vi "Read MR8888 File.vi"(11 "Path":path=path "D:/同步空间/曲线生成/原始曲线/8、记录仪MR8888--AUTO0001.csv") -> (3 "Data Series":T1[](array[typedef]))   [LabVIEW 2020, in "Data Viewer.lvlib"]
uses:
  Data Viewer.lvlib
  Data Serie--cluster.ctl
  File Type--enum.ctl
  45ada8d8-9367-42c1-a51c-dab00799f42c.vi
  4505f498-e49c-4e88-80e6-bc2a5fe8a2a1.vi
  1e224d21-03f6-4504-93f9-5a21471556d5.vi
  2c9b7013-6681-49c9-91fb-dfb68bc23b96.vi
  <vilib>/Utility/file.llb/Read Delimited Spreadsheet (string).vi
  <vilib>/Comparison/Equal/Equal Functor/Equal Functor.lvclass
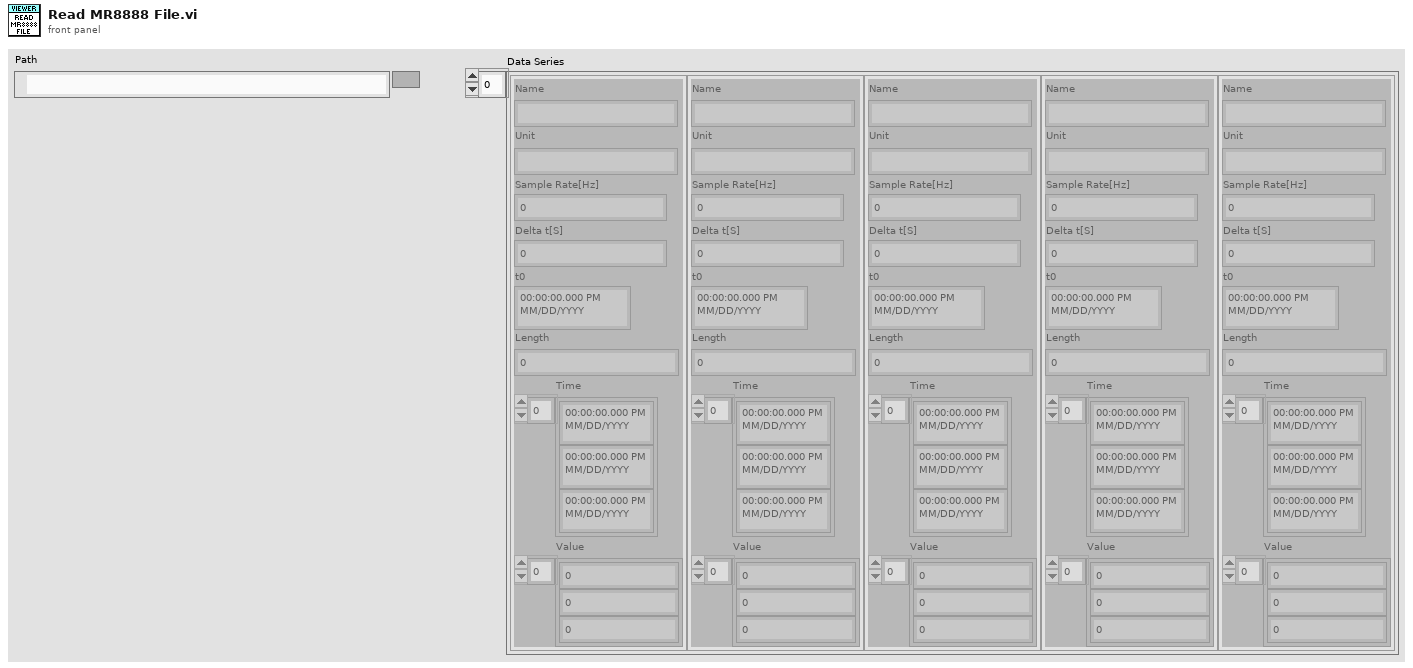
[diagram p1: front panel]
types:
  T1 = typedef "Data Viewer.lvlib/Data Serie--cluster.ctl" = cluster{"Name":string, "Unit":string, "Sample Rate[Hz]":dbl, "Delta t[S]":dbl, "t0":timestamp, "Length":i32, "Time":timestamp[], "Value":dbl[]}
  T2 = typedef "Data Viewer.lvlib/File Type--enum.ctl" = enum16{"伟思环境箱", "增达环境箱", "广五所环境箱", "无纸记录仪", "帕捷SA00339", "记录仪840", "记录仪8400", "记录仪MR888", "*.csv"}
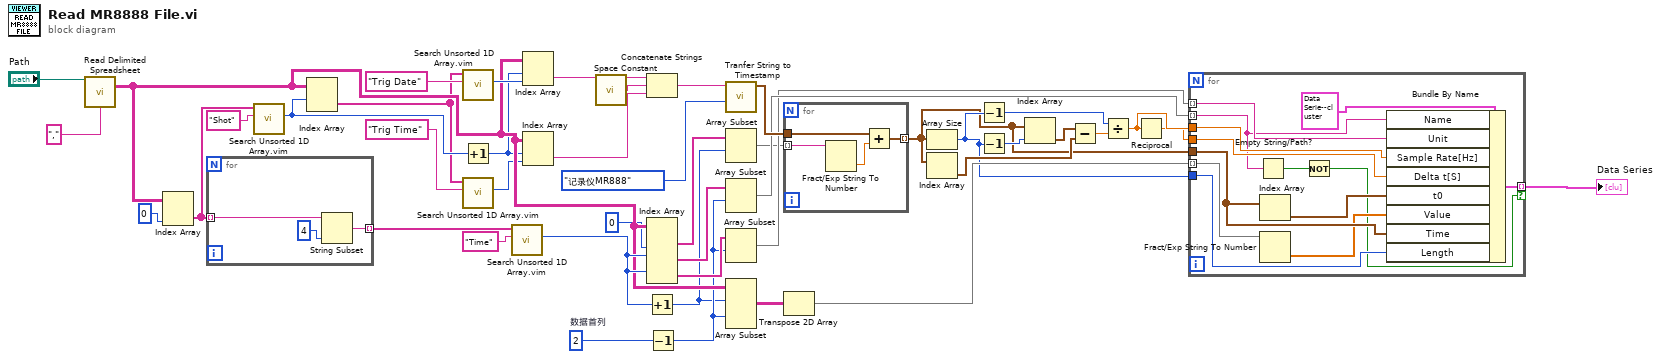
[diagram p0: block diagram]
diagram:
  w18 = 2  # 数据首列
  n1 = call-poly <vilib>:"Read Delimited Spreadsheet.vi"("file path (dialog if empty)"="Path", "delimiter (\\t)"="," ("delimiter (\\t)")) -> ("all rows"=w31:string[][])  [unwired: 8 in, 5 out]
  n2 = Index Array(array=w31, index (col)=0 ("disabled index (col)")) -> (element=w36:string[])  [unwired: 1 in]
  n3 = for {
    tunnel: w36 -> [w47] mode=indexing
    tunnel: [w45] -> w35 mode=indexing
    n4 = String Subset(string=w47, length (rest)=4 ("length (rest)")) -> (substring=w45:string)  [unwired: 1 in]
  }
  n5 = call "Search Unsorted 1D Array.vim"("element"="Shot", "unsorted 1D array"=w36) -> ("index of element"=w33:i32)  [unwired: 9 in]
  n6 = Index Array(array=w31, index (row)=w33) -> (element=w28:string[])  [unwired: 1 in]
  n7 = call "Search Unsorted 1D Array.vim"("element"="Trig Date", "unsorted 1D array"=w28) -> ("index of element"=w32:i32)  [unwired: 9 in]
  n8 = Increment(x=w33) -> (x+1=w30:i32)
  n9 = call "Search Unsorted 1D Array.vim"("element"="Trig Time", "unsorted 1D array"=w28) -> ("index of element"=w27:i32)  [unwired: 9 in]
  n10 = call "Search Unsorted 1D Array.vim"("element"="Time", "unsorted 1D array"=w35) -> ("index of element"=w40:i32)  [unwired: 9 in]
  n11 = Index Array(array=w31, index (row)=w30, index (col)=w32) -> (element=w26:string)
  n12 = Index Array(array=w31, index (row)=w30, index (col)=w27) -> (element=w25:string)
  n13 = call <vilib>:"Space Constant.vi"() -> ("String"=w24:string)
  n14 = Concatenate Strings(w26, w24, w25) -> (w23:string)
  n15 = Index Array(array=w31, index (col) #1=0 ("disabled index (col)"), index (row) #2=w40, index (row) #3=w40) -> (element #1=w21:string[], element #2=w20:string[], element #3=w19:string[])  [unwired: 3 in]
  n16 = Increment(x=w40) -> (x+1=w3:i32)
  n17 = Decrement(x=w18) -> (x-1=w6:i32)
  n18 = call "Tranfer String to Timestamp.vi"("File Type"=File_Type--enum."记录仪MR888", "String"=w23) -> ("time stamp"=w37:timestamp)  [unwired: 9 in]
  n19 = Array Subset(array=w21, index=w3) -> (w2:string[])  [unwired: 1 in]
  n20 = Array Subset(array=w20, index=w6) -> (w16:string[])  [unwired: 1 in]
  n21 = Array Subset(array=w19, index=w6) -> (w15:string[])  [unwired: 1 in]
  n22 = Array Subset(array=w31, index (row)=w3, index (col)=w6) -> (w17:string[][])  [unwired: 2 in]
  n23 = for {
    tunnel: w2 -> [w49] mode=indexing
    tunnel: w37 -> [w51]
    tunnel: [w50] -> w1 mode=indexing
    n24 = Fract/Exp String To Number(string=w49) -> (number=w48:dbl)  [unwired: 3 in, 1 out]
    n25 = Add(x=w51, y=w48) -> (x+y=w50:timestamp)
  }
  n26 = Transpose 2D Array(2D array=w17) -> (transposed array=w14:string[][])
  n27 = Array Size(array=w1) -> (size(s)=w4:i32)
  n28 = Index Array(array=w1) -> (element=w11:timestamp)  [unwired: 1 in]
  n29 = Decrement(x=w4) -> (x-1=w5:i32)
  n30 = Decrement(x=w4) -> (x-1=w13:i32)
  n31 = Index Array(array=w1, index=w13) -> (element=w12:timestamp)
  n32 = Subtract(x=w12, y=w11) -> (x-y=w10:dbl)
  n33 = Divide(x=w5, y=w10) -> (x/y=w9:dbl)
  n34 = Reciprocal(x=w9) -> (1/x=w8:dbl)
  n35 = for {
    tunnel: w16 -> [w54] mode=indexing
    tunnel: w15 -> [w56] mode=indexing
    tunnel: w14 -> [w61] mode=indexing
    tunnel: w1 -> [w62]
    tunnel: w9 -> [w59]
    tunnel: w8 -> [w58]
    tunnel: [w57] -> w7 mode=indexing if=w52
    tunnel: w4 -> [w55]
    n36 = Empty String/Path?(string/path=w54) -> (empty?=w53:bool)
    n37 = Index Array(array=w62) -> (element=w63:timestamp)  [unwired: 1 in]
    n38 = Fract/Exp String To Number(string=w61) -> (number=w60:dbl[])  [unwired: 3 in, 1 out]
    n39 = Not(x=w53) -> (.not. x?=w52:bool)
    n40 = Bundle By Name(cluster=T1 {"Name"="", "Unit"="", "Sample Rate[Hz]"=0.0, "Delta t[S]"=0.0, "t0"=timestamp(0 s since 1904-01-01), "Length"=0, "Time"=[], "Value"=[]} ("Data Serie"), "Name"=w54, "Unit"=w56, "Sample Rate[Hz]"=w59, "Delta t[S]"=w58, "t0"=w63, "Value"=w60, "Time"=w62, "Length"=w55) -> (w57:T1)
  }
  "Data Series" <- w7
